vi "Read GL840 File.vi"(11 "Path":path=path "D:/同步空间/曲线生成/原始曲线/6、记录仪840--240617-084400_Converted_CP1.csv") -> (3 "Data Series":T1[](array[typedef]))   [LabVIEW 2020, in "Data Viewer.lvlib"]
uses:
  Data Viewer.lvlib
  Data Serie--cluster.ctl
  File Type--enum.ctl
  7bfe4985-3a25-4a87-b238-63f0ca83d9b9.vi
  4505f498-e49c-4e88-80e6-bc2a5fe8a2a1.vi
  45ada8d8-9367-42c1-a51c-dab00799f42c.vi
  <vilib>/Utility/file.llb/Read Delimited Spreadsheet (string).vi
  <vilib>/Comparison/Equal/Equal Functor/Equal Functor.lvclass
  <vilib>/regexp/Match Regular Expression.xnode
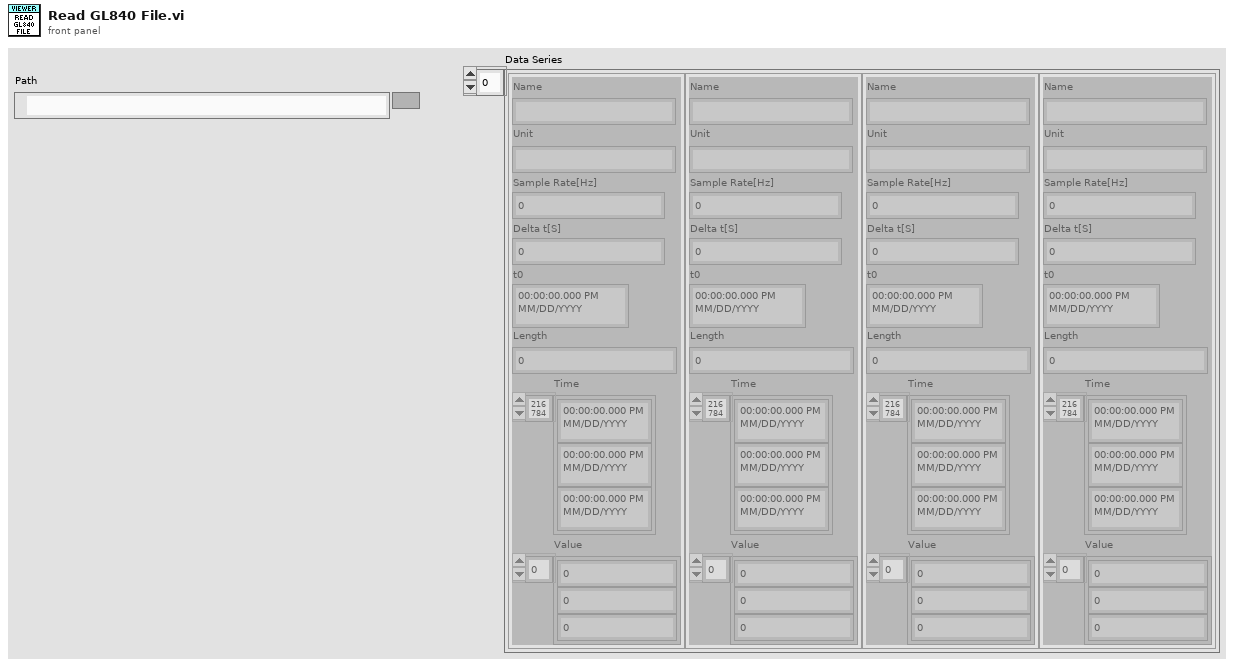
[diagram p1: front panel]
types:
  T1 = typedef "Data Viewer.lvlib/Data Serie--cluster.ctl" = cluster{"Name":string, "Unit":string, "Sample Rate[Hz]":dbl, "Delta t[S]":dbl, "t0":timestamp, "Length":i32, "Time":timestamp[], "Value":dbl[]}
  T2 = typedef "Data Viewer.lvlib/File Type--enum.ctl" = enum16{"伟思环境箱", "增达环境箱", "广五所环境箱", "无纸记录仪", "帕捷SA00339", "记录仪840", "记录仪8400", "记录仪MR888", "*.csv"}
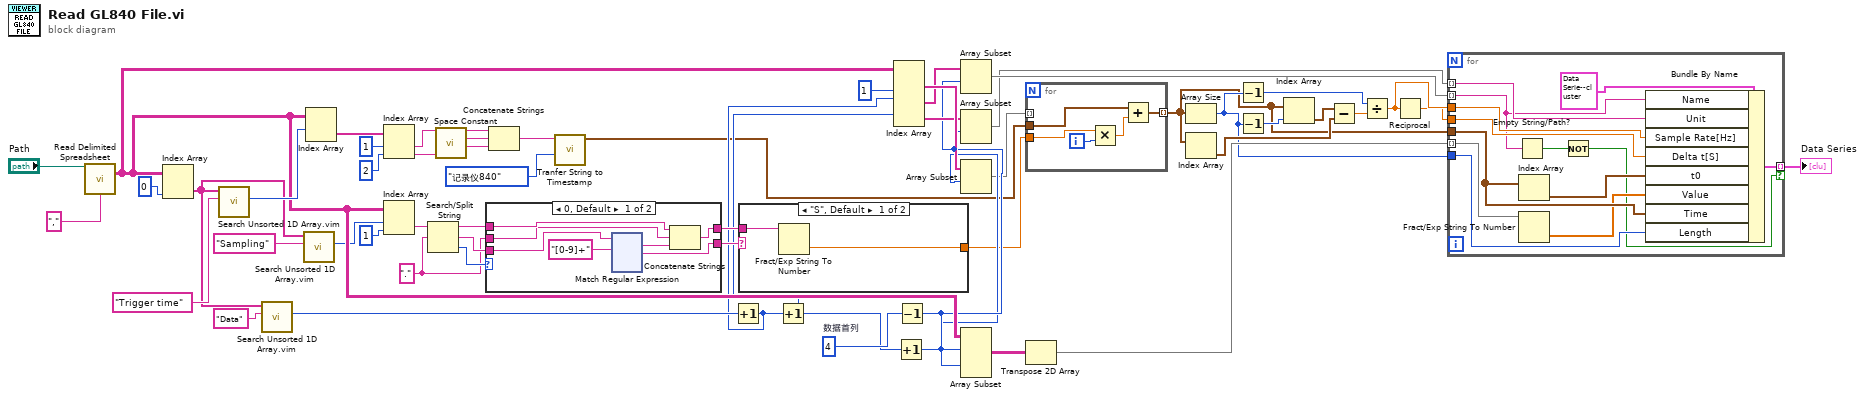
[diagram p0: block diagram]
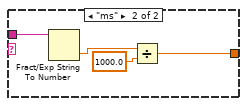
[diagram p2: hidden frame]
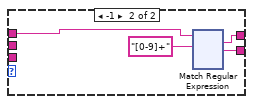
[diagram p3: hidden frame]
diagram:
  w22 = 4  # 数据首列
  w32 = "." ("search string/char (-)")
  n1 = call-poly <vilib>:"Read Delimited Spreadsheet.vi"("file path (dialog if empty)"="Path", "delimiter (\\t)"="," ("delimiter (\\t)")) -> ("all rows"=w38:string[][])  [unwired: 8 in, 5 out]
  n2 = Index Array(array=w38, index (col)=0 ("disabled index (col)")) -> (element=w39:string[])  [unwired: 1 in]
  n3 = call "Search Unsorted 1D Array.vim"("element"="Trigger time", "unsorted 1D array"=w39) -> ("index of element"=w47:i32)  [unwired: 9 in]
  n4 = call "Search Unsorted 1D Array.vim"("element"="Data", "unsorted 1D array"=w39) -> ("index of element"=w49:i32)  [unwired: 9 in]
  n5 = call "Search Unsorted 1D Array.vim"("element"="Sampling", "unsorted 1D array"=w39) -> ("index of element"=w37:i32)  [unwired: 9 in]
  n6 = Index Array(array=w38, index (row)=w47) -> (element=w46:string[])  [unwired: 1 in]
  n7 = Index Array(array=w46, index #1=1 ("index"), index #2=2 ("index")) -> (element #1=w43:string, element #2=w41:string)
  n8 = Index Array(array=w38, index (row)=w37, index (col)=1 ("disabled index (col)")) -> (element=w31:string)
  n9 = Search/Split String(string=w31, search string/char (-)=w32) -> (substring before match=w34:string, match + rest of string=w33:string, offset of match=w35:i32)  [unwired: 1 in]
  n10 = call <vilib>:"Space Constant.vi"() -> ("String"=w42:string)
  n11 = case shown="0, Default" w35 {
    tunnel: [w54 w177] -> w29
    tunnel: [w58 w176] -> w30
    tunnel: w34 -> [w57 w175]
    tunnel: w33 -> [w59 _]
    tunnel: w32 -> [w56 _]
    frame 0, Default {
      n12 = xnode "Match Regular Expression"("input string"=w59, "regular expression"="[0-9]+") -> ("whole match"=w55:string, "after match"=w58:string)  [unwired: 4 in, 3 out]
      n13 = Concatenate Strings(w57, w56, w55) -> (w54:string)
    }
    frame -1 {
      n14 = xnode "Match Regular Expression"("input string"=w175, "regular expression"="[0-9]+") -> ("whole match"=w177:string, "after match"=w176:string)  [unwired: 4 in, 3 out]
    }
  }
  n15 = Concatenate Strings(w43, w42, w41) -> (w28:string)
  n16 = call "Tranfer String to Timestamp.vi"("File Type"=File_Type--enum."记录仪840", "String"=w28) -> ("time stamp"=w3:timestamp)  [unwired: 9 in]
  n17 = Increment(x=w49) -> (x+1=w7:i32)
  n18 = case shown="\"S\", Default" w30 {
    tunnel: w29 -> [w294 w298]
    tunnel: [w293 w295] -> w2
    frame "S", Default {
      n19 = Fract/Exp String To Number(string=w294) -> (number=w293:dbl)  [unwired: 3 in, 1 out]
    }
    frame "ms" {
      n20 = Fract/Exp String To Number(string=w298) -> (number=w297:dbl)  [unwired: 3 in, 1 out]
      n21 = Divide(x=w297, y=1000.0) -> (x/y=w295:dbl)
    }
  }
  n22 = Increment(x=w7) -> (x+1=w6:i32)
  n23 = Index Array(array=w38, index (col) #1=1 ("disabled index (col)"), index (row) #2=w7, index (row) #3=w6) -> (element #1=w25:string[], element #2=w24:string[], element #3=w23:string[])  [unwired: 3 in]
  n24 = Increment(x=w6) -> (x+1=w5:i32)
  n25 = Decrement(x=w22) -> (x-1=w10:i32)
  n26 = Array Subset(array=w24, index=w10) -> (w20:string[])  [unwired: 1 in]
  n27 = Array Subset(array=w23, index=w10) -> (w19:string[])  [unwired: 1 in]
  n28 = Array Subset(array=w25, index=w5) -> (w4:string[])  [unwired: 1 in]
  n29 = Array Subset(array=w38, index (row)=w5, index (col)=w10) -> (w21:string[][])  [unwired: 2 in]
  n30 = for {
    tunnel: w4 -> [_] mode=indexing
    tunnel: w3 -> [w301]
    tunnel: w2 -> [w303]
    tunnel: [w299] -> w1 mode=indexing
    i -> [w302]
    n31 = Multiply(x=w303, y=w302) -> (x*y=w300:dbl)
    n32 = Add(x=w301, y=w300) -> (x+y=w299:timestamp)
  }
  n33 = Transpose 2D Array(2D array=w21) -> (transposed array=w18:string[][])
  n34 = Array Size(array=w1) -> (size(s)=w8:i32)
  n35 = Index Array(array=w1) -> (element=w15:timestamp)  [unwired: 1 in]
  n36 = Decrement(x=w8) -> (x-1=w9:i32)
  n37 = Decrement(x=w8) -> (x-1=w17:i32)
  n38 = Index Array(array=w1, index=w17) -> (element=w16:timestamp)
  n39 = Subtract(x=w16, y=w15) -> (x-y=w14:dbl)
  n40 = Divide(x=w9, y=w14) -> (x/y=w13:dbl)
  n41 = Reciprocal(x=w13) -> (1/x=w12:dbl)
  n42 = for {
    tunnel: w20 -> [w305] mode=indexing
    tunnel: w19 -> [w308] mode=indexing
    tunnel: w18 -> [w313] mode=indexing
    tunnel: w1 -> [w314]
    tunnel: w13 -> [w311]
    tunnel: w12 -> [w310]
    tunnel: [w309] -> w11 mode=indexing if=w304
    tunnel: w8 -> [w307]
    n43 = Empty String/Path?(string/path=w305) -> (empty?=w306:bool)
    n44 = Index Array(array=w314) -> (element=w315:timestamp)  [unwired: 1 in]
    n45 = Fract/Exp String To Number(string=w313) -> (number=w312:dbl[])  [unwired: 3 in, 1 out]
    n46 = Not(x=w306) -> (.not. x?=w304:bool)
    n47 = Bundle By Name(cluster=T1 {"Name"="", "Unit"="", "Sample Rate[Hz]"=0.0, "Delta t[S]"=0.0, "t0"=timestamp(0 s since 1904-01-01), "Length"=0, "Time"=[], "Value"=[]} ("Data Serie"), "Name"=w305, "Unit"=w308, "Sample Rate[Hz]"=w311, "Delta t[S]"=w310, "t0"=w315, "Value"=w312, "Time"=w314, "Length"=w307) -> (w309:T1)
  }
  "Data Series" <- w11
